vi "Own20261012_DeleteFormulaParameter.vi"() -> ()   [LabVIEW 2024]
panel:
  out "error out":errorcluster caption="错误输出"
  in  "parameter_id":u32
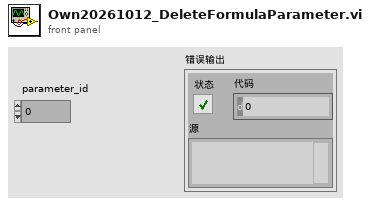
[diagram p1: front panel]
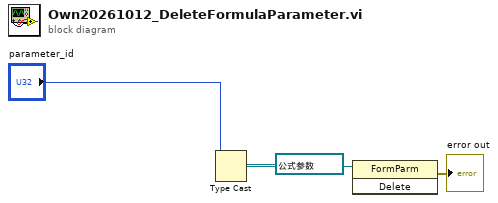
[diagram p0: block diagram]
diagram:
  n1 = Type Cast(type=refnum<vi> refnum ("引用"), x="parameter_id") -> (*(type *) &x=w2:refnum<vi>)
  n2 = invoke class="FormParm" method="Delete"(reference=w2) -> (error out=→"error out":errorcluster)  [unwired: 2 in, 2 out]
